vi "Build ATM Message.vi"(8 "error in":errorcluster, 9 "Amount":dbl, 10 "Account":T1, 11 "Message Type":T2) -> (0 "error out":errorcluster, 3 "ATM Message":string)   [LabVIEW 2026]
doc: "Builds the text the ATM shows on its display for one Message Type. Main Menu takes the customer name from Account, Balance Inquiry the balance from Account, and Deposit Complete / Withdrawal Complete the money value from Amount. Money is formatted with a dollar sign and two decimals, always with a period as decimal separator. Pure string building: no file or user interface access.\n\nError behaviour: if error in carries an error, nothing is built, ATM Message is empty and the error is passed to error out unchanged."
uses:
  Controls/ATM Message Type.ctl
  Controls/ATM Account.ctl
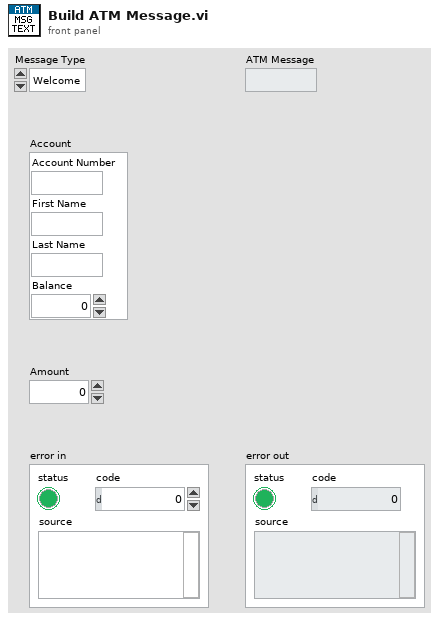
[diagram p1: front panel]
types:
  T1 = typedef "ATM Account.ctl" = cluster{"Account Number":string, "First Name":string, "Last Name":string, "Balance":dbl}
  T2 = typedef "ATM Message Type.ctl" = enum16{"Welcome", "Main Menu", "Account Verification Failed", "Session Terminate", "Deposit", "Deposit Complete", "Withdrawal", "Withdrawal Complete", "Withdrawal Failed", "Balance Inquiry"}
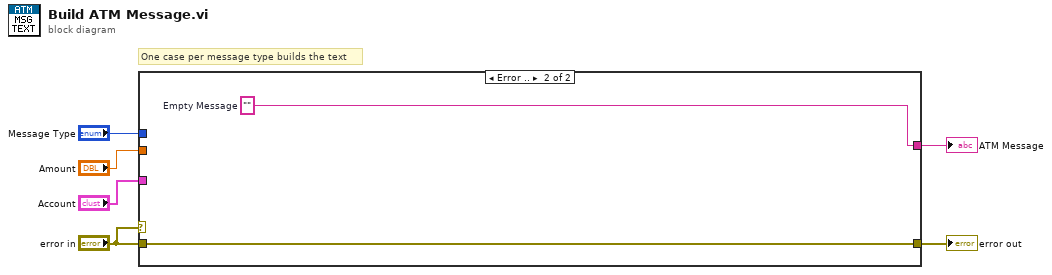
[diagram p0: block diagram]
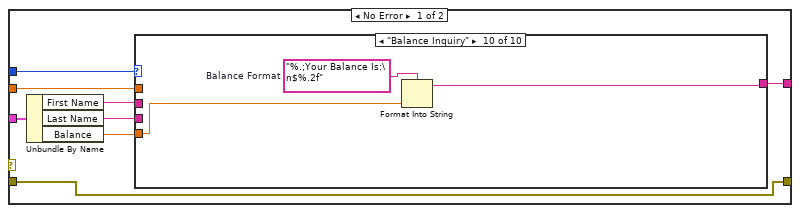
[diagram p2: hidden frame]
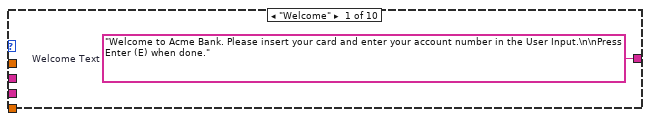
[diagram p3: hidden frame]
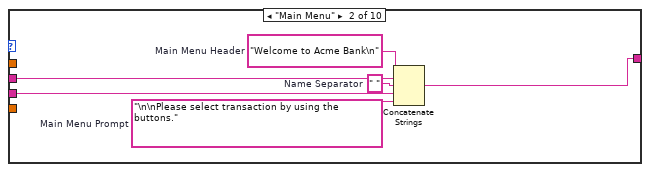
[diagram p4: hidden frame]
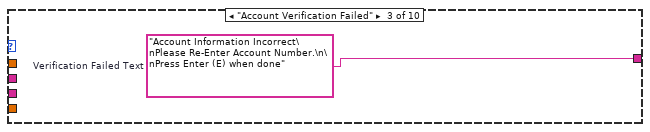
[diagram p5: hidden frame]
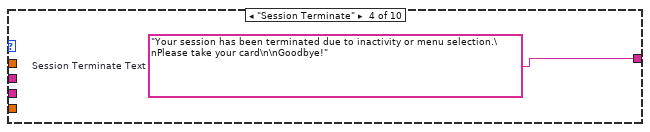
[diagram p6: hidden frame]
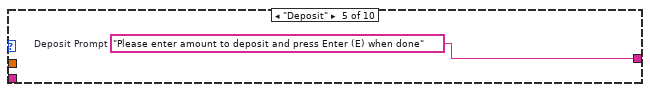
[diagram p7: hidden frame]
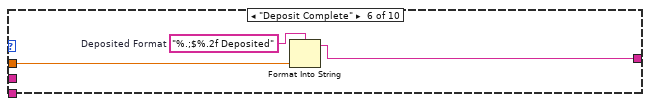
[diagram p8: hidden frame]
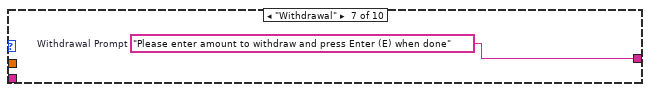
[diagram p9: hidden frame]
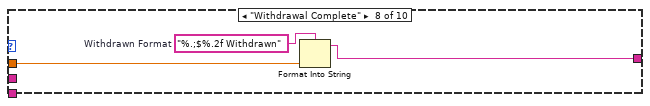
[diagram p10: hidden frame]
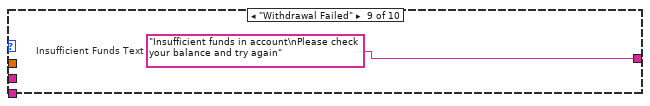
[diagram p11: hidden frame]
diagram:
  # "One case per message type builds the text"
  n1 = case shown="Error .." "error in" {
    tunnel: "error in" -> [w7 w36]
    tunnel: "Message Type" -> [w9 _]
    tunnel: "Account" -> [w14 _]
    tunnel: "Amount" -> [w10 _]
    tunnel: [w8 w37] -> w2
    tunnel: [w7 w36] -> w1
    frame No Error {
      n2 = Unbundle By Name(w14) -> ("First Name"=w13:string, "Last Name"=w12:string, "Balance"=w11:dbl)
      n3 = case shown="\"Balance Inquiry\"" w9 {
        tunnel: w13 -> [_ w20 _ _ _ _ _ _ _ _]
        tunnel: w12 -> [_ w18 _ _ _ _ _ _ _ _]
        tunnel: w11 -> [_ _ _ _ _ _ _ _ _ w35]
        tunnel: w10 -> [_ _ _ _ _ w27 _ w31 _ _]
        tunnel: [w15 w16 w22 w23 w24 w25 w28 w29 w32 w33] -> w8
        frame "Welcome" {
          w15 = "Welcome to Acme Bank. Please insert your card and enter your account number in the User Input.\n\nPress Enter (E) when done."  # Welcome Text
        }
        frame "Main Menu" {
          w17 = "\n\nPlease select transaction by using the buttons."  # Main Menu Prompt
          w19 = " "  # Name Separator
          w21 = "Welcome to Acme Bank\n"  # Main Menu Header
          n4 = Concatenate Strings(w21, w20, w19, w18, w17) -> (w16:string)
        }
        frame "Account Verification Failed" {
          w22 = "Account Information Incorrect\nPlease Re-Enter Account Number.\n\nPress Enter (E) when done"  # Verification Failed Text
        }
        frame "Session Terminate" {
          w23 = "Your session has been terminated due to inactivity or menu selection.\nPlease take your card\n\nGoodbye!"  # Session Terminate Text
        }
        frame "Deposit" {
          w24 = "Please enter amount to deposit and press Enter (E) when done"  # Deposit Prompt
        }
        frame "Deposit Complete" {
          w26 = "%.;$%.2f Deposited"  # Deposited Format
          n5 = Format Into String(format string=w26, w27) -> (resulting string=w25:string)  [unwired: 2 in, 1 out]
        }
        frame "Withdrawal" {
          w28 = "Please enter amount to withdraw and press Enter (E) when done"  # Withdrawal Prompt
        }
        frame "Withdrawal Complete" {
          w30 = "%.;$%.2f Withdrawn"  # Withdrawn Format
          n6 = Format Into String(format string=w30, w31) -> (resulting string=w29:string)  [unwired: 2 in, 1 out]
        }
        frame "Withdrawal Failed" {
          w32 = "Insufficient funds in account\nPlease check your balance and try again"  # Insufficient Funds Text
        }
        frame "Balance Inquiry" {
          w34 = "%.;Your Balance Is:\n$%.2f"  # Balance Format
          n7 = Format Into String(format string=w34, w35) -> (resulting string=w33:string)  [unwired: 2 in, 1 out]
        }
      }
    }
    frame Error {
      w37 = ""  # Empty Message
    }
  }
  "ATM Message" <- w2
  "error out" <- w1
